vi "Example 02d - Coroutines.vi"() -> ()   [LabVIEW 2020]
uses:
  Lua for LabVIEW/Lua Thread/Lua Thread.lvclass
  C:/Users/Nicholas Folse/Documents/workspace/github-tauterra.llc/Lua for LabVIEW/Lua for LabVIEW/Lua/Lua.lvclass
  Lua for LabVIEW/Lua/Lua.lvclass
panel:
  in  "stop after n iters":i32=4
  out "yielded indicies":i64[](array[numeric])
  in  "count":i64=10
  out "error out":errorcluster
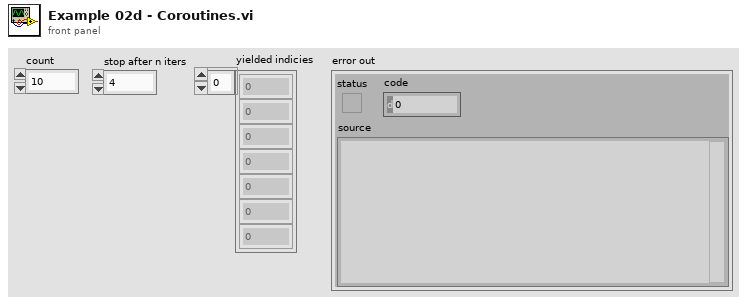
[diagram p1: front panel]
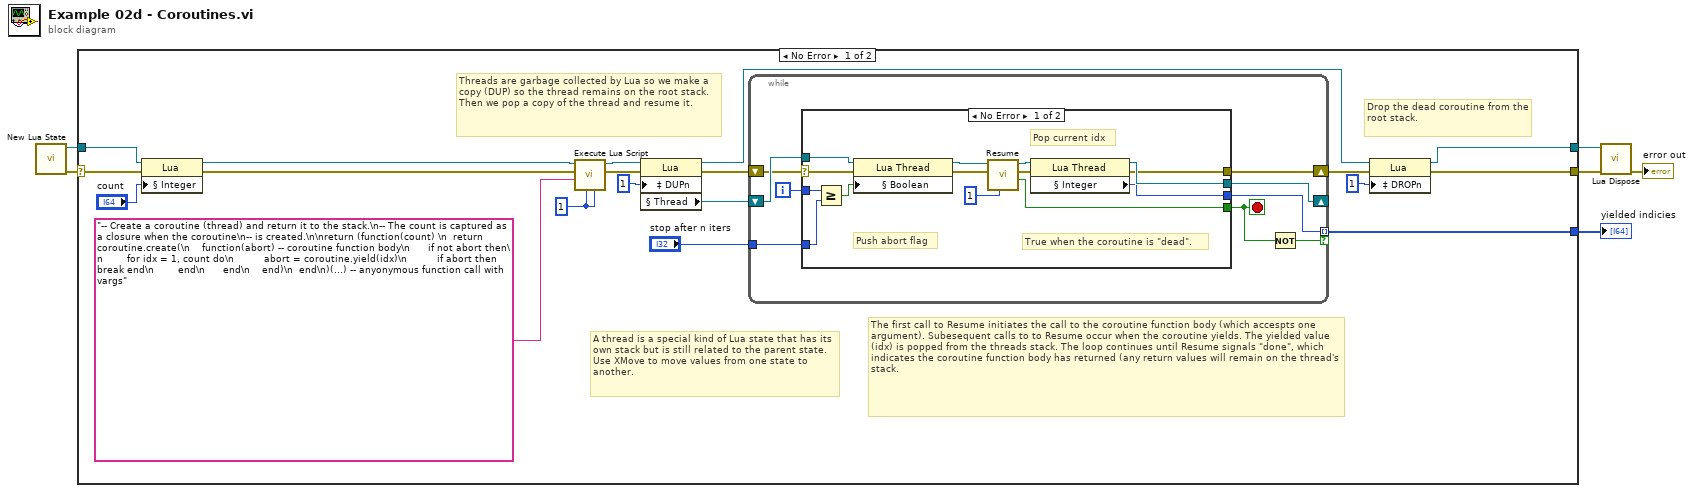
[diagram p0: block diagram]
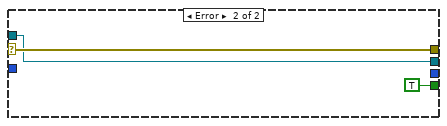
[diagram p2: hidden frame]
diagram:
  n1 = call "New Lua State.vi"() -> ("error out"=w2:errorcluster, "Lua out"=w6:refnum<class "Lua.lvclass">)  [unwired: 10 in]
  n2 = case shown="No Error" w2 {
    selector: w2 -> [w16 w52]
    tunnel: [w7 w52] -> w1
    tunnel: [w8 w53] -> w5
    tunnel: w6 -> [w18 w53]
    tunnel: [w24 _] -> w4
    frame No Error {
      w9 = 1 ("nargs")
      # "The first call to Resume initiates the call to the coroutine function body (which accespts one argument). Subesequent calls to to Resume occur when the coroutine yields. The yielded value (idx) is popped from the threads stack. The loop continues until Resume signals \"done\", which indicates the coroutine function body has returned (any return values will remain on the thread's stack."
      # "Drop the dead coroutine from the root stack."
      # "Threads are garbage collected by Lua so we make a copy (DUP) so the thread remains on the root stack. Then we pop a copy of the thread and resume it."
      # "A thread is a special kind of Lua state that has its own stack but is still related to the parent state. Use XMove to move values from one state to another."
      n3 = property class="Lua"(reference=w18, error in=w16, "§ Integer"="count") -> (reference out=w17:refnum<class "Lua.lvclass">, error out=w12:errorcluster)
      n4 = call-dynamic "Execute Lua Script.vi"("nresults"=w9, "nargs"=w9, "lua script"="-- Create a coroutine (thread) and return it to the stack.\n-- The count is captured as a closure when the coroutine\n-- is created.\n\nreturn (function(count) \n  return coroutine.create(\n    function(abort) -- coroutine function body\n      if not abort then\n        for idx = 1, count do\n          abort = coroutine.yield(idx)\n          if abort then break end\n        end\n      end\n    end)\n  end\n)(...) -- anyonymous function call with vargs", "error in (no error)"=w12, "Lua in"=w17) -> ("error out"=w10:errorcluster, "Lua out"=w23:refnum<class "Lua.lvclass">)  [unwired: 5 in]
      n5 = property class="Lua"(reference=w23, error in=w10, "‡ DUPn"=1) -> (reference out=w19:refnum<class "Lua.lvclass">, error out=w15:errorcluster, "§ Thread"=w22:refnum<class "Lua Thread.lvclass">)
      n6 = while {
        shift-right: [w33] -> w25
        shift-left: w15 -> [w30]
        shift-right: [w34] -> _
        shift-left: w22 -> [w31]
        tunnel: [w32] -> w24 mode=indexing if=w28
        tunnel: "stop after n iters" -> [w26]
        i -> [w27]
        stop <- w29 stop-if-true
        n7 = case shown="No Error" w30 {
          selector: w30 -> [w35 w51]
          tunnel: [w48 w49] -> w34
          tunnel: [w47 w51] -> w33
          tunnel: [w46 _] -> w32
          tunnel: [w44 TRUE] -> w29
          tunnel: w31 -> [w40 w49]
          tunnel: w27 -> [w43 _]
          tunnel: w26 -> [w42 _]
          frame No Error {
            # "True when the coroutine is \"dead\"."
            # "Pop current idx"
            # "Push abort flag"
            n8 = Greater Or Equal?(x=w43, y=w42) -> (x >= y?=w39:bool)
            n9 = property class="Lua Thread"(reference=w40, error in=w35, "§ Boolean"=w39) -> (reference out=w38:refnum<class "Lua Thread.lvclass">, error out=w37:errorcluster)
            n10 = call-dynamic "Resume.vi"("nargs"=1, "error in (no error)"=w37, "Lua Thread in"=w38) -> ("done?"=w44:bool, "error out"=w36:errorcluster, "Lua Thread out"=w45:refnum<class "Lua Thread.lvclass">)  [unwired: 5 in, 1 out]
            n11 = property class="Lua Thread"(reference=w45, error in=w36) -> (reference out=w48:refnum<class "Lua Thread.lvclass">, error out=w47:errorcluster, "§ Integer"=w46:i64)
          }
          frame Error {
          }
        }
        n12 = Not(x=w29) -> (.not. x?=w28:bool)
      }
      n13 = property class="Lua"(reference=w19, error in=w25, "‡ DROPn"=1) -> (reference out=w8:refnum<class "Lua.lvclass">, error out=w7:errorcluster)
    }
    frame Error {
    }
  }
  "yielded indicies" <- w4
  n14 = call-dynamic "Lua Dispose.vi"("error in (no error)"=w1, "Lua in"=w5) -> ("error out"=→"error out":errorcluster)  [unwired: 9 in]
